vi "test reply 2.vi"(8 "error in (no error)":errorcluster, 10 "Numeric":dbl, 11 "Abstract DAQ Triggered Actor in":refnum<class "Abstract DAQ Triggered Actor.lvclass">) -> (0 "error out":errorcluster, 2 "Numeric 2":dbl, 3 "Abstract DAQ Triggered Actor out":refnum<class "Abstract DAQ Triggered Actor.lvclass">)   [LabVIEW 2020, in "DAQ Timed SPIM.lvlib" / "Abstract DAQ Triggered Actor.lvlib" / "Abstract DAQ Triggered Actor.lvclass"]
uses:
  Abstract DAQ Triggered Actor.lvclass
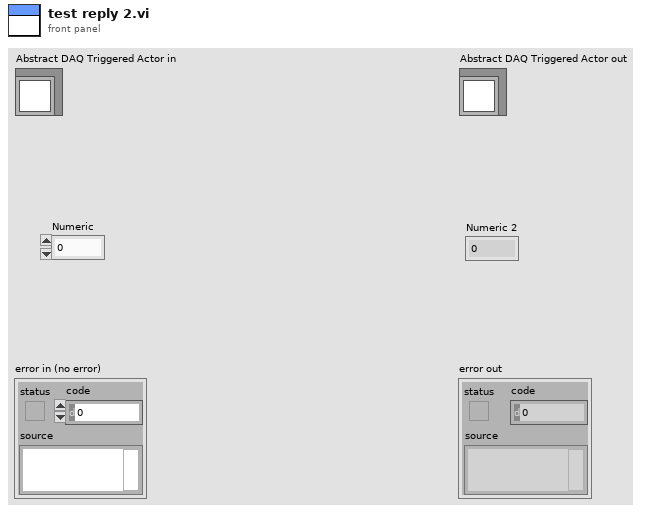
[diagram p1: front panel]
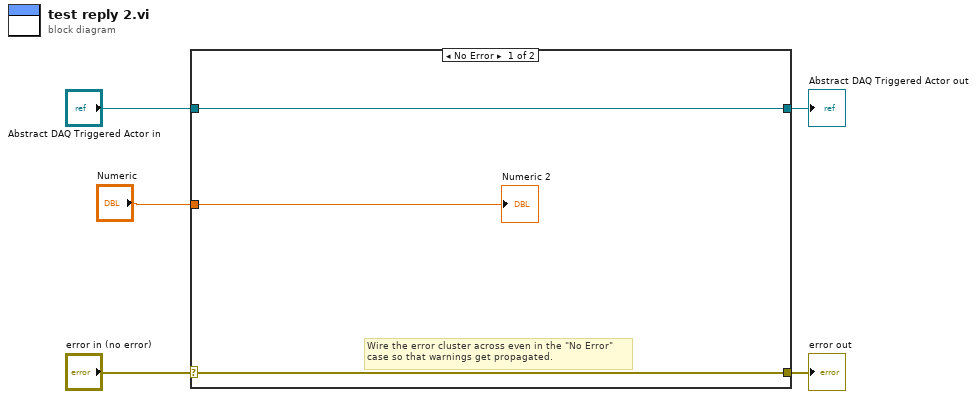
[diagram p0: block diagram]
diagram:
  n1 = case shown="No Error" "error in (no error)" {
    selector: "error in (no error)" -> [w7 w10]
    tunnel: [w7 w10] -> w4
    tunnel: [w8 w9] -> w2
    tunnel: "Abstract DAQ Triggered Actor in" -> [w8 w9]
    tunnel: "Numeric" -> [w6 _]
    frame No Error {
      # "Wire the error cluster across even in the \"No Error\"\ncase so that warnings get propagated."
      "Numeric 2" <- w6
    }
    frame Error {
    }
  }
  "error out" <- w4
  "Abstract DAQ Triggered Actor out" <- w2
